vi "UDP Receiver.vi"() -> ()   [LabVIEW 2026]
panel:
  out "Numeric 2":dbl
  out "String 4":string
  out "String 3":string
  in  "Blank Button":bool
  in  "Numeric":i32
  in  "String 2":string
  in  "String":string
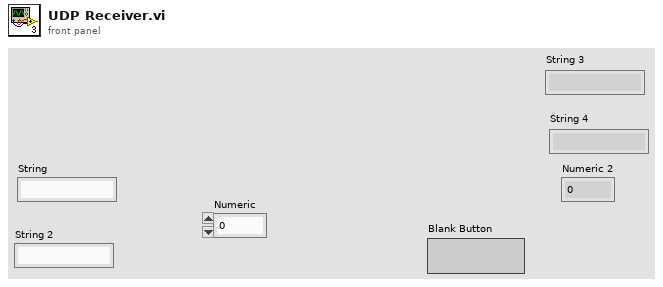
[diagram p1: front panel]
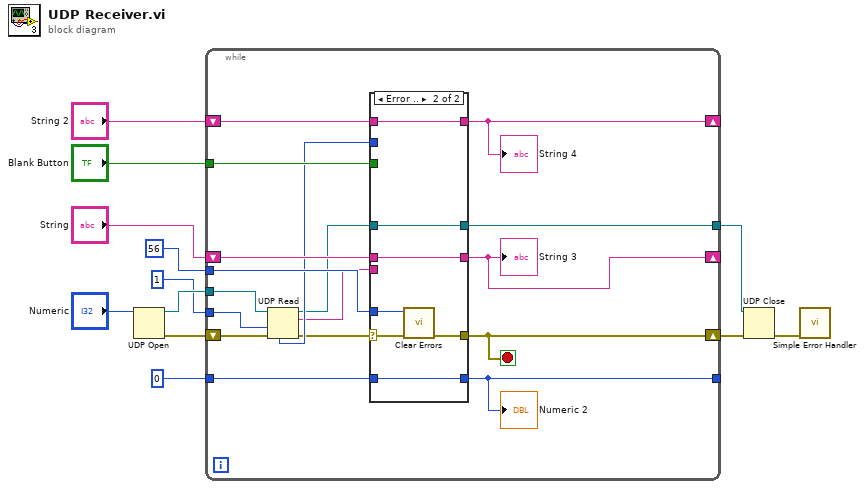
[diagram p0: block diagram]
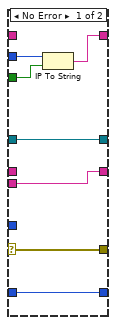
[diagram p2: hidden frame]
diagram:
  n1 = UDP Open(11:"Numeric") -> (port=w10:refnum<k16>, 0:w9:errorcluster)  [unwired: 4 in, 1 out]
  n2 = while {
    tunnel: 56 -> [w29]
    tunnel: w10 -> [w28]
    shift-right: [w19] -> w8
    shift-left: w9 -> [w27]
    shift-right: [w15] -> _
    shift-left: "String" -> [w26]
    shift-right: [w14] -> _
    shift-left: "String 2" -> [w25]
    tunnel: "Blank Button" -> [w24]
    tunnel: [w20] -> w4
    tunnel: 0 -> [w16]
    tunnel: 1 -> [w17]
    tunnel: [w13] -> _
    stop <- w19 stop-if-true
    n3 = UDP Read(connection ID=w28, timeout ms (25000)=w17, 8:w27) -> (data out=w22:string, error out=w18:errorcluster, 3:w21:refnum<k16>, 6:w23:u32)  [unwired: 1 in, 1 out]
    n4 = case shown="Error .." w18 {
      selector: w18 -> [w31 w38]
      tunnel: w29 -> [_ w41]
      tunnel: w26 -> [_ w42]
      tunnel: w25 -> [_ w43]
      tunnel: [w34 w43] -> w14
      tunnel: [w33 w42] -> w15
      tunnel: w24 -> [w36 _]
      tunnel: w23 -> [w35 _]
      tunnel: w22 -> [w33 _]
      tunnel: w21 -> [w32 w39]
      tunnel: [w32 w39] -> w20
      tunnel: [w31 w40] -> w19
      tunnel: w16 -> [w30 w37]
      tunnel: [w30 w37] -> w13
      frame No Error {
        n5 = IP To String(1:w36, 2:w35) -> (0:w34:string)
      }
      frame Error {
        n6 = call <vilib>:"Clear Errors.vi"("error in (no error)"=w38, "specific error code to clear (0: all)"=w41) -> ("error out"=w40:errorcluster)  [unwired: 4 in, 1 out]
      }
    }
    "String 3" <- w15
    "String 4" <- w14
    "Numeric 2" <- w13
  }
  n7 = UDP Close(connection ID=w4, 8:w8) -> (error out=w1:errorcluster)  [unwired: 1 out]
  n8 = call <vilib>:"Simple Error Handler.vi"("error in (no error)"=w1) -> ()  [unwired: 4 in, 5 out]
